vi "Build Step Table.vi"(10 "Step Results":T1[](array[typedef]), 11 "Sequence File":T2) -> (3 "Step Table":string[][](array[string]))   [LabVIEW 2026]
doc: "Builds the step table for display: one row per step of the Sequence File with columns Step, Name, Command, Setpoints, Conditions, Dwell ms, Timeout ms, Result, Measured, Target, Duration ms, Reason. Setpoints is one 'channel=value' entry per setpoint joined with '; '; Conditions is one 'channel target+/-tolerance' entry per condition joined with '; '. Result, Measured, Target and Duration ms come from the Step Result at the same index; a step without a result shows empty result text and zeros. Pure function, no error terminals, AF-free."
uses:
  Typedefs/Sequence File.ctl
  Typedefs/Step Config.ctl
  Typedefs/Channel Value.ctl
  Typedefs/Condition.ctl
  Typedefs/Step Result.ctl
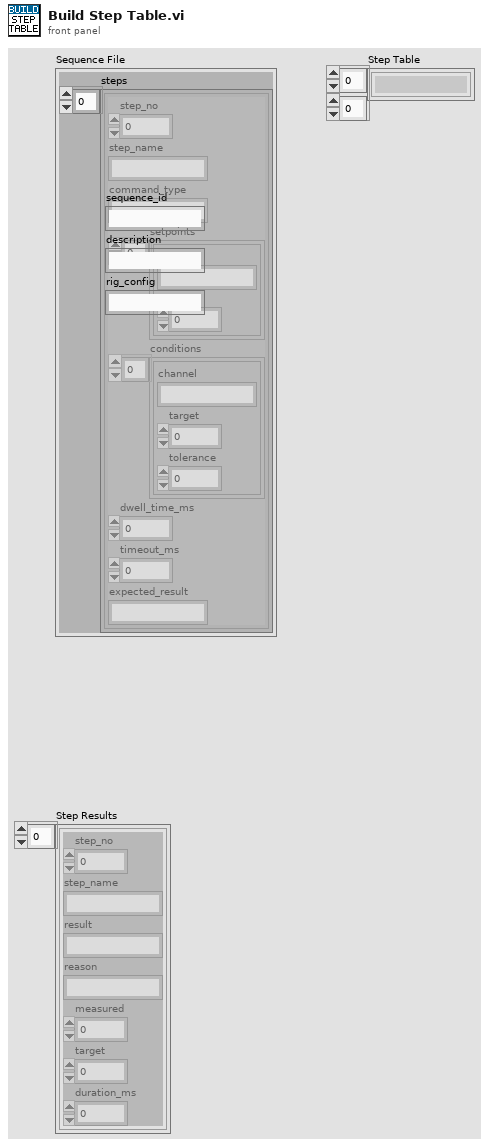
[diagram p1: front panel]
types:
  T1 = typedef "Step Result.ctl" = cluster{"step_no":i32, "step_name":string, "result":string, "reason":string, "measured":dbl, "target":dbl, "duration_ms":dbl}
  T2 = typedef "Sequence File.ctl" = cluster{"sequence_id":string, "description":string, "rig_config":string, "steps":T3[]}
  T3 = typedef "Step Config.ctl" = cluster{"step_no":i32, "step_name":string, "command_type":string, "setpoints":T4[], "conditions":T5[], "dwell_time_ms":i32, "timeout_ms":i32, "expected_result":string}
  T4 = typedef "Channel Value.ctl" = cluster{"channel":string, "value":dbl}
  T5 = typedef "Condition.ctl" = cluster{"channel":string, "target":dbl, "tolerance":dbl}
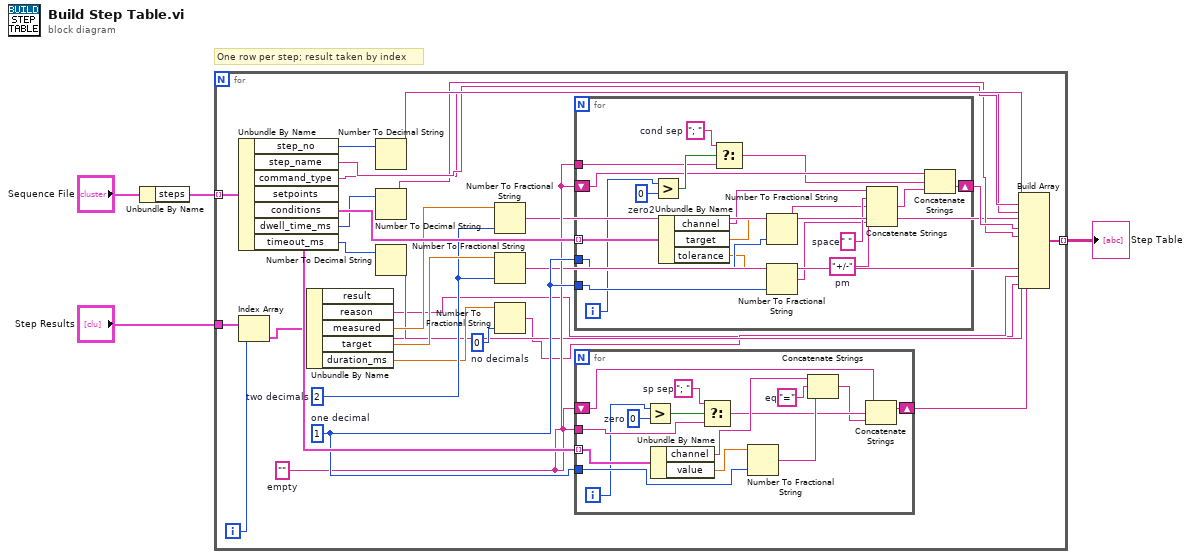
[diagram p0: block diagram]
diagram:
  # "One row per step; result taken by index"
  n1 = Unbundle By Name("Sequence File") -> ("steps"=w3:T3[])
  n2 = for {
    tunnel: w3 -> [w33] mode=indexing
    tunnel: "Step Results" -> [w28]
    tunnel: [w6] -> w1 mode=indexing
    i -> [w5]
    w29 = ""  # empty
    w30 = 1  # one decimal
    w19 = 0  # no decimals
    w21 = 2  # two decimals
    n3 = Unbundle By Name(w33) -> ("step_no"=w26:i32, "step_name"=w17:string, "command_type"=w16:string, "setpoints"=w32:T4[], "conditions"=w31:T5[], "dwell_time_ms"=w25:i32, "timeout_ms"=w24:i32)
    n4 = Index Array(array=w28, index=w5) -> (element=w27:T1)
    n5 = Unbundle By Name(w27) -> ("result"=w11:string, "reason"=w7:string, "measured"=w23:dbl, "target"=w22:dbl, "duration_ms"=w20:dbl)
    n6 = Number To Decimal String(number=w26) -> (decimal integer string=w18:string)  [unwired: 1 in]
    n7 = Number To Decimal String(number=w25) -> (decimal integer string=w13:string)  [unwired: 1 in]
    n8 = Number To Decimal String(number=w24) -> (decimal integer string=w12:string)  [unwired: 1 in]
    n9 = Number To Fractional String(number=w23, precision (6)=w21) -> (F-format string=w10:string)  [unwired: 2 in]
    n10 = Number To Fractional String(number=w22, precision (6)=w21) -> (F-format string=w9:string)  [unwired: 2 in]
    n11 = Number To Fractional String(number=w20, precision (6)=w19) -> (F-format string=w8:string)  [unwired: 2 in]
    n12 = for {
      tunnel: w31 -> [w52] mode=indexing
      shift-right: [w35] -> w14
      shift-left: w29 -> [w38]
      tunnel: w30 -> [w50]
      tunnel: w30 -> [w48]
      tunnel: w29 -> [w39]
      i -> [w34]
      w42 = 0  # zero2
      w41 = "; "  # cond sep
      w44 = "+/-"  # pm
      w46 = " "  # space
      n13 = Greater?(x=w34, y=w42) -> (0:w40:bool)
      n14 = Unbundle By Name(w52) -> ("channel"=w47:string, "target"=w51:dbl, "tolerance"=w49:dbl)
      n15 = Select(t=w41, s=w40, f=w39) -> (s? t:f=w37:string)
      n16 = Number To Fractional String(number=w51, precision (6)=w50) -> (F-format string=w45:string)  [unwired: 2 in]
      n17 = Number To Fractional String(number=w49, precision (6)=w48) -> (F-format string=w43:string)  [unwired: 2 in]
      n18 = Concatenate Strings(w47, w46, w45, w44, w43) -> (w36:string)
      n19 = Concatenate Strings(w38, w37, w36) -> (w35:string)
    }
    n20 = for {
      tunnel: w32 -> [w67] mode=indexing
      shift-right: [w54] -> w15
      shift-left: w29 -> [w57]
      tunnel: w30 -> [w65]
      tunnel: w29 -> [w58]
      i -> [w53]
      w61 = 0  # zero
      w60 = "; "  # sp sep
      w63 = "="  # eq
      n21 = Greater?(x=w53, y=w61) -> (0:w59:bool)
      n22 = Unbundle By Name(w67) -> ("channel"=w64:string, "value"=w66:dbl)
      n23 = Select(t=w60, s=w59, f=w58) -> (s? t:f=w56:string)
      n24 = Number To Fractional String(number=w66, precision (6)=w65) -> (F-format string=w62:string)  [unwired: 2 in]
      n25 = Concatenate Strings(w64, w63, w62) -> (w55:string)
      n26 = Concatenate Strings(w57, w56, w55) -> (w54:string)
    }
    n27 = Build Array(w18, w17, w16, w15, w14, w13, w12, w11, w10, w9, w8, w7) -> (w6:string[])
  }
  "Step Table" <- w1
